vi "GetCurrentProcessId Wrapper Template.vi"(11 "error in":errorcluster) -> (4 "process ID":u32, 15 "error out":errorcluster)   [LabVIEW 2020]
doc: "Returns the identifier of the calling process - LabVIEW itself - through kernel32.dll GetCurrentProcessId (stdcall, called in any thread). Compare it with user32 GetWindowThreadProcessId.vi to tell LabVIEW's own windows from everybody else's. When error in carries an error the DLL is not called. Generated by scripts\\Build Win32 Wrappers.vi - do not edit by hand, rebuild it."
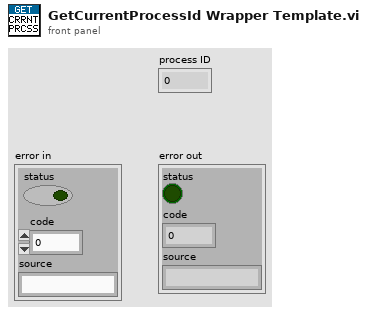
[diagram p1: front panel]
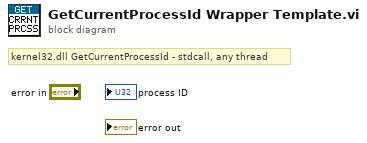
[diagram p0: block diagram]
diagram:
  # "kernel32.dll GetCurrentProcessId - stdcall, any thread"
